vi "Emergency Stop.vi"(8 "error in":errorcluster, 11 "Sequence Executor in":refnum<class "Sequence Executor.lvclass">) -> (0 "error out":errorcluster, 3 "Sequence Executor out":refnum<class "Sequence Executor.lvclass">)   [LabVIEW 2026, in "Sequence Executor.lvclass"]
doc: "Emergency stop: Abort Sequence with reason E-STOP. Message: Emergency Stop Msg (sent at High priority)."
uses:
  Sequence Executor.lvclass
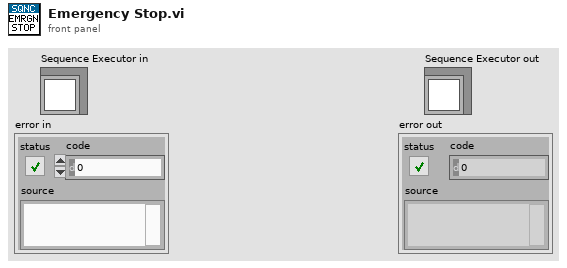
[diagram p1: front panel]
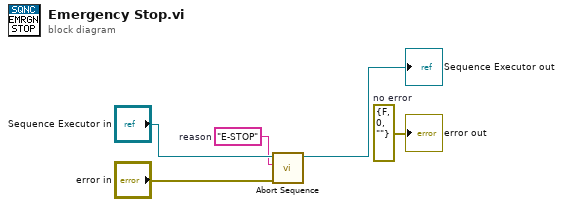
[diagram p0: block diagram]
diagram:
  w4 = "E-STOP"  # reason
  w1 = errorcluster {"status"=FALSE, "code"=0, "source"=""}  # no error
  n1 = call "Abort Sequence.vi"("error in"="error in", "reason"=w4, "Sequence Executor in"="Sequence Executor in") -> ("Sequence Executor out"=→"Sequence Executor out":refnum<class "Sequence Executor.lvclass">)  [unwired: 7 in, 1 out]
  "error out" <- w1
